vi "Get Error Description & Source.vi"(9 "error in (no error)":errorcluster) -> (2 "error source":string, 3 "error description":string)   [LabVIEW 2019, in "Error Generation.lvlib"]
doc: "- - -\nCopyright (c) 2023, Merecs Engineering GmbH"
uses:
  Error Generation.lvlib
panel:
  # "Connector Pane"
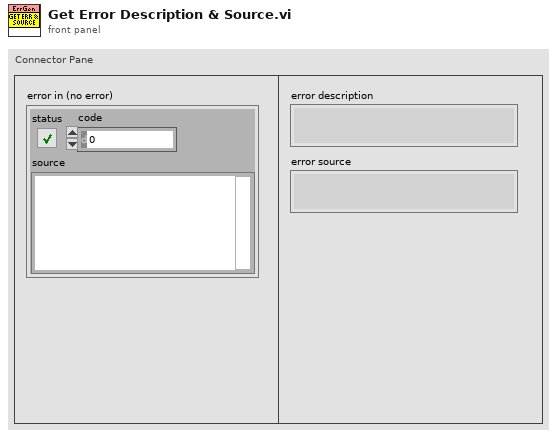
[diagram p1: front panel]
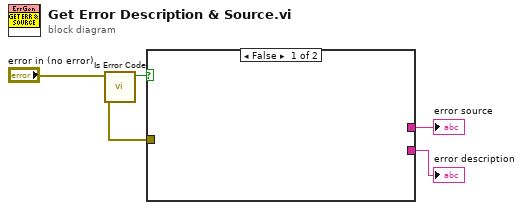
[diagram p0: block diagram]
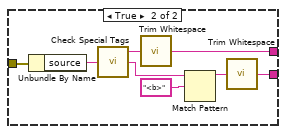
[diagram p2: hidden frame]
diagram:
  n1 = call "Is Error Code.vi"("error in (no error)"="error in (no error)") -> ("Code!=0"=w3:bool)  [unwired: 5 in, 1 out]
  n2 = case shown="False" w3 {
    tunnel: "error in (no error)" -> [_ w12]
    tunnel: [_ w6] -> w2
    tunnel: [_ w5] -> w1
    frame False {
    }
    frame True {
      n3 = Unbundle By Name(w12) -> ("source"=w11:string)
      n4 = call <vilib>:"Check Special Tags.vi"("source"=w11) -> ("Before Tag (source)"=w10:string, "After Tag (special data)"=w8:string)  [unwired: 1 out]
      n5 = call <vilib>:"Trim Whitespace.vi"("string"=w10) -> ("trimmed string"=w6:string)  [unwired: 1 in]
      n6 = Match Pattern(string=w8, regular expression="<b>") -> (before substring=w7:string)  [unwired: 1 in, 3 out]
      n7 = call <vilib>:"Trim Whitespace.vi"("string"=w7) -> ("trimmed string"=w5:string)  [unwired: 1 in]
    }
  }
  "error description" <- w1
  "error source" <- w2
